vi "while loop.vi"() -> ()   [LabVIEW 2018]
panel:
  out "Tank":dbl(slide) scale=0.0..150.0
  out "i":i32
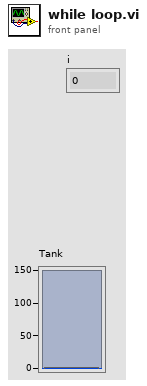
[diagram p1: front panel]
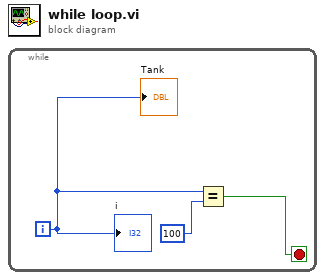
[diagram p0: block diagram]
diagram:
  n1 = while {
    i -> [w3]
    stop <- w1 stop-if-true
    n2 = Equal?(x=w3, y=100) -> (x = y?=w1:bool)
    "i" <- w3
    "Tank" <- w3
  }
